vi "Read Server Info.vi"(8 "error in":errorcluster, 9 "parameters":string[][](array[string]), 10 "id in":i32, 11 "read?":bool) -> (0 "error out":errorcluster, 1 "capabilities":string, 2 "_meta":string, 3 "serverInfo":string)   [LabVIEW 2020, in "MCP Server.lvlib"]
doc: "Reads serverInfo and capabilities as initialize reports them, by calling initialize.vi with a synthetic initialize request, so that a modern (MCP 2026-07-28) result always names the same server as initialize. Used by Complete Modern MCP Result.vi.\n\nserverInfo is {\"name\":..,\"version\":..}, _meta is {\"io.modelcontextprotocol/serverInfo\":<serverInfo>} and capabilities is the JSON object of result.capabilities. initialize.vi is only called when read? is TRUE; otherwise the outputs carry no data.\n\nRuns regardless of error in, which is passed through unchanged; the JSONtext errors are not passed on."
uses:
  MCP Server.lvlib
  <vilib>/JDP Science/JSONtext/Next JSON Value.vi
  <vilib>/JDP Science/JSONtext/String Subset.vi
  <vilib>/JDP Science/JSONtext/Parsing/Advance past next JSON Value (inlined COPY).vi
  <vilib>/JDP Science/JSONtext/Parsing/Advance past whitespace.vi
  <vilib>/JDP Science/JSONtext/Parsing/Advance past String.vi
  <vilib>/JDP Science/JSONtext/Parsing/Advance past Number.vi
  <vilib>/JDP Science/JSONtext/Parsing/Advance past Line Ending.vi
  <vilib>/JDP Science/JSONtext/Parsing/Parse Full Path or Item Name.vi
  <vilib>/JDP Science/JSONtext/Parsing/Advance past Array.vi
  <vilib>/JDP Science/JSONtext/Parsing/Advance past Object.vi
  <vilib>/JDP Science/JSONtext/support/Error Cluster From Code.vi
  <vilib>/JDP Science/JSONtext/Offset/Find Item Locations by Path.vi
  <vilib>/JDP Science/JSONtext/JSONtext.lvlib
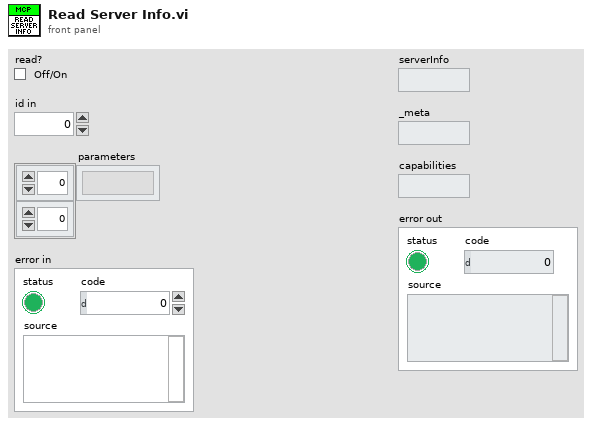
[diagram p1: front panel]
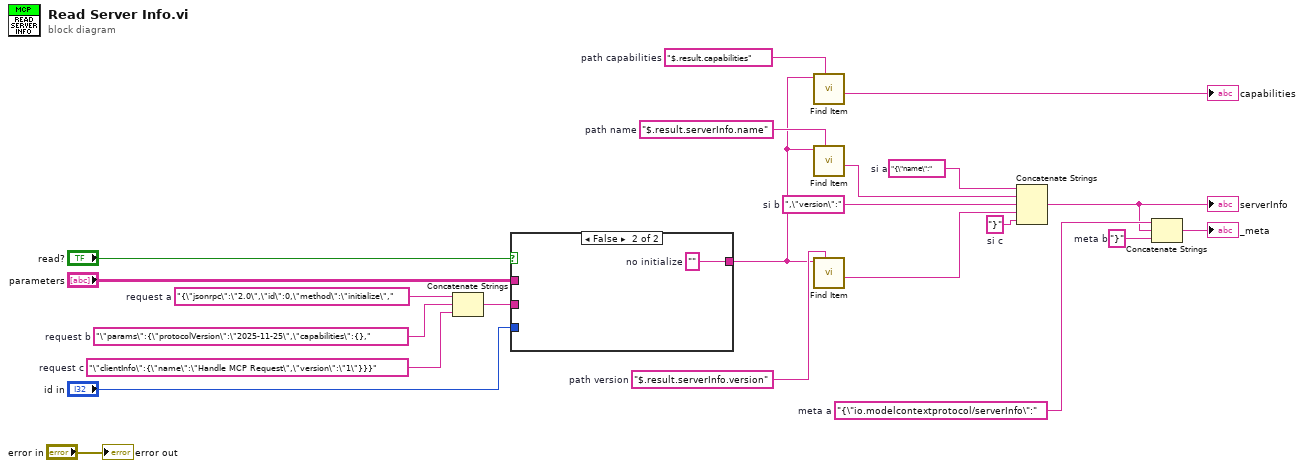
[diagram p0: block diagram]
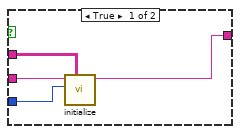
[diagram p2: hidden frame]
diagram:
  w5 = "}"  # meta b
  w6 = "{\"io.modelcontextprotocol/serverInfo\":"  # meta a
  w7 = "}"  # si c
  w9 = ",\"version\":"  # si b
  w11 = "{\"name\":"  # si a
  w13 = "$.result.capabilities"  # path capabilities
  w14 = "$.result.serverInfo.version"  # path version
  w15 = "$.result.serverInfo.name"  # path name
  w20 = "\"clientInfo\":{\"name\":\"Handle MCP Request\",\"version\":\"1\"}}}"  # request c
  w21 = "\"params\":{\"protocolVersion\":\"2025-11-25\",\"capabilities\":{},"  # request b
  w22 = "{\"jsonrpc\":\"2.0\",\"id\":0,\"method\":\"initialize\","  # request a
  n1 = Concatenate Strings(w22, w21, w20) -> (w19:string)
  n2 = case shown="False" "read?" {
    tunnel: w19 -> [w24 _]
    tunnel: "id in" -> [w25 _]
    tunnel: "parameters" -> [w26 _]
    tunnel: [w23 w27] -> w12
    frame True {
      n3 = call "initialize.vi"("parameters"=w26, "server id"=w25, "message json"=w24) -> ("response"=w23:string)  [unwired: 7 in, 1 out]
    }
    frame False {
      w27 = ""  # no initialize
    }
  }
  n4 = call <vilib>:"Find Item.vi"("$Path or Item Name"=w13, "JSON"=w12) -> ("<JSON>"=→"capabilities":string)  [unwired: 6 in, 3 out]
  n5 = call <vilib>:"Find Item.vi"("$Path or Item Name"=w15, "JSON"=w12) -> ("<JSON>"=w10:string)  [unwired: 6 in, 3 out]
  n6 = call <vilib>:"Find Item.vi"("$Path or Item Name"=w14, "JSON"=w12) -> ("<JSON>"=w8:string)  [unwired: 6 in, 3 out]
  n7 = Concatenate Strings(w11, w10, w9, w8, w7) -> (w4:string)
  "serverInfo" <- w4
  n8 = Concatenate Strings(w6, w4, w5) -> (→"_meta":string)
  "error out" <- "error in"
